vi "Get Devices.vi"(6 "timeout (ms)":i32=5000, 8 "error in":errorcluster, 10 "Refresh Device List":bool, 11 "gRPC ID":T2) -> (0 "error out":errorcluster, 2 "devices":T1[](array[typedef]), 3 "gRPC ID out":T2)   [LabVIEW 2021, in "CAN_Writer_NIXNET_Wrapper.lvlib"]
uses:
  CAN_Writer_NIXNET_Wrapper.lvlib
  <vilib>/gRPC/LabVIEW gRPC Library/Shared/grpcId.ctl
  CanWriterNixnet_client/CanWriterNixnet_client.lvlib
  CanWriterNixnet_client/RPC Messages/cif_can_writer_nixnet_RefreshDevices.ctl
  <vilib>/gRPC/LabVIEW gRPC Library/grpc-lvsupport-release.lvlib
  CanWriterNixnet_client/RPC Messages/cif_can_writer_nixnet_XnetDevice.ctl
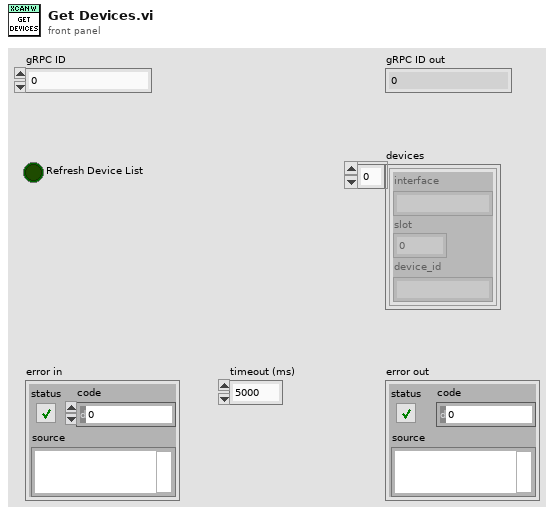
[diagram p1: front panel]
types:
  T1 = typedef "CanWriterNixnet_client.lvlib/cif_can_writer_nixnet_XnetDevice.ctl" = cluster{"interface":string, "slot":u32, "device_id":string}
  T2 = typedef "grpc-lvsupport-release.lvlib/grpcId.ctl" = u64
  T3 = typedef "CanWriterNixnet_client.lvlib/cif_can_writer_nixnet_RefreshDevices.ctl" = cluster{"refresh_device_list":bool}
  T4 = typedef "CanWriterNixnet_client.lvlib/cif_can_writer_nixnet_XnetDevices.ctl" = cluster{"devices":T1[]}
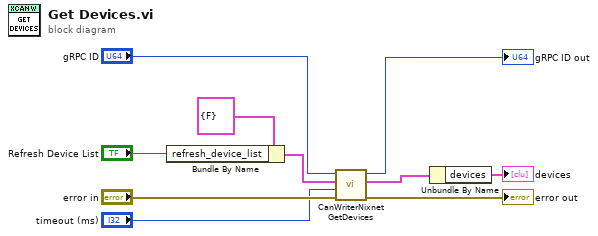
[diagram p0: block diagram]
diagram:
  n1 = Bundle By Name(cluster=T3 {"refresh_device_list"=FALSE} ("Request Data"), "refresh_device_list"="Refresh Device List") -> (w1:T3)
  n2 = call "CanWriterNixnet GetDevices.vi"("error in"="error in", "timeout (ms)"="timeout (ms)", "Request Data"=w1, "gRPC ID"="gRPC ID") -> ("error out"=→"error out":errorcluster, "Response Data"=w8:T4, "gRPC ID out"=→"gRPC ID out":T2)  [unwired: 5 in]
  n3 = Unbundle By Name(w8) -> ("devices"=→"devices":T1[])
